vi "Data to JSON.vi"(8 "error in (no error)":errorcluster, 10 "Data in":variant) -> (0 "error out":errorcluster, 1 "<JSON> data":string, 2 "<JSON> header":string)   [LabVIEW 2019, in "XPUB.lvclass"]
uses:
  XPUB.lvclass
  <vilib>/LabVIEW Open Source Project/Epoch Date & Time/formatter.iso8601/Seconds Units -- enum.ctl
  813cc443-dbb8-45a6-9550-6b12cca50f99.vi
  <vilib>/JDP Science/JSONtext/Variant to JSON Text.vi
  <vilib>/JDP Science/JSONtext/LVClass Serializer/JSONtext LVClass Serializer.lvclass
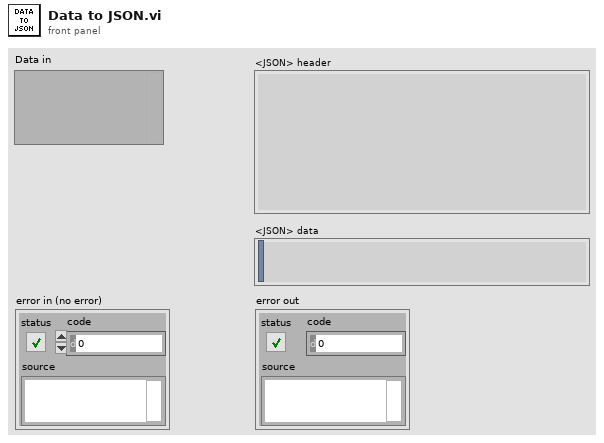
[diagram p1: front panel]
types:
  T1 = typedef "Seconds Units -- enum.ctl" = enum16{"second", "millisecond", "microsecond", "nanosecond"}
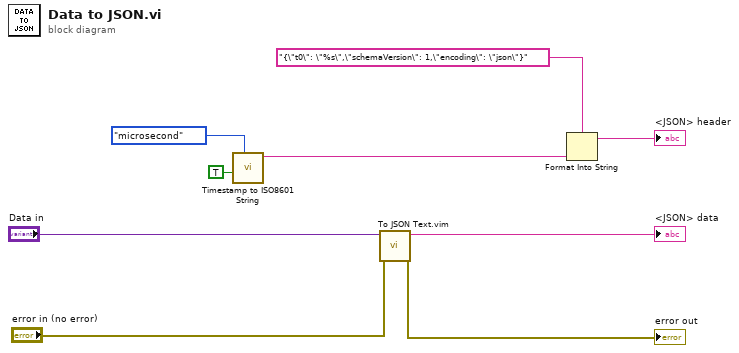
[diagram p0: block diagram]
diagram:
  n1 = call <vilib>:"Timestamp to ISO8601 String.vi"("Unit (ms)"=Seconds_Units_--_enum."microsecond", "UTC? (F)"=TRUE) -> ("ISO8601 String"=w7:string)  [unwired: 9 in]
  n2 = call "To JSON Text.vim"("error in (no error)"="error in (no error)", "Anything"="Data in") -> ("error out"=→"error out":errorcluster, "<JSON>"=→"<JSON> data":string)  [unwired: 8 in]
  n3 = Format Into String(format string="{\"t0\": \"%s\",\"schemaVersion\": 1,\"encoding\": \"json\"}", w7) -> (resulting string=→"<JSON> header":string)  [unwired: 2 in, 1 out]
